vi "validate line configuration.vi"(7 "modbus":refnum<class "Modbus Module configuration.lvclass">, 11 "line in":T1) -> (1 "valid?":bool, 2 "issues":string, 3 "line out":T1)   [LabVIEW 2015, in "Modbus Module editor node.lvclass"]
doc: "Validate that Line In is a valid Modbus line and can be added to existing Configuration In without any conflicts.\n\nPlatypus Framework 1.0.1.65\nNI Systems Engineering - National Instruments"
uses:
  Modbus Module editor node.lvclass
  table line.ctl
  module/module channel/Modbus Module Channel.lvclass
  module/configuration/Modbus Module configuration.lvclass
  module/configuration/Modbus Module configuration.lvclass/Modbus Module configuration.ctl
  <vilib>/NI/Tag Bus/tag/tag descriptor.lvclass/tag descriptor.ctl
  module/module channel/Modbus Module Channel.lvclass/Modbus Module Channel.ctl
  <vilib>/NI/Tag Bus/tag/Data Type.ctl
  <vilib>/NI/Tag Bus/tag/read tag name.vi
  module/module channel/Read modbus type.vi
  module/module channel/Read starting address.vi
  <vilib>/NI/Tag Bus/tag/read data type.vi
  module/module channel/Read subindex (bool).vi
  <vilib>/NI/Tag Bus/tag/tag descriptor.lvclass
  <vilib>/NI/Tag Bus Module Framework/module configuration/TBM module configuration.lvclass
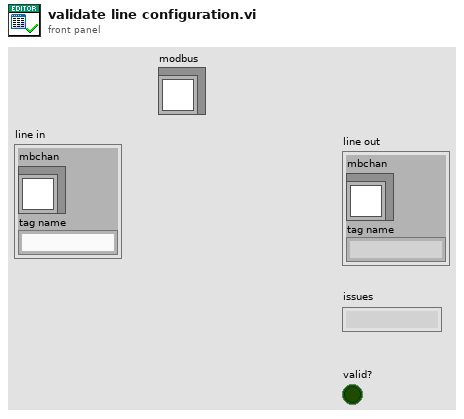
[diagram p1: front panel]
types:
  T1 = typedef "Modbus Module editor node.lvclass/table line.ctl" = cluster{"mbchan":refnum<class "Modbus Module Channel.lvclass">, "tag name":string}
  T2 = typedef "tag bus.lvlib/tag descriptor.lvclass/Data Type.ctl" = enum16{"Double", "Single", "I64", "I32", "I16", "I8", "U64", "U32", "U16", "U8", "Boolean", "String", "Array of Double", "Array of Single", "Array of I64", "Array of I32", "Array of I16", "Array of I8", "Array of U64", "Array of U32", "Array of U16", "Array of U8", "Array of Boolean", "Array of String"}
  T3 = typedef "Modbus Module Channel.lvclass/data bank type.ctl" = enum16{"Coils", "Discrete Inputs", "Input Registers", "Holding Registers"}
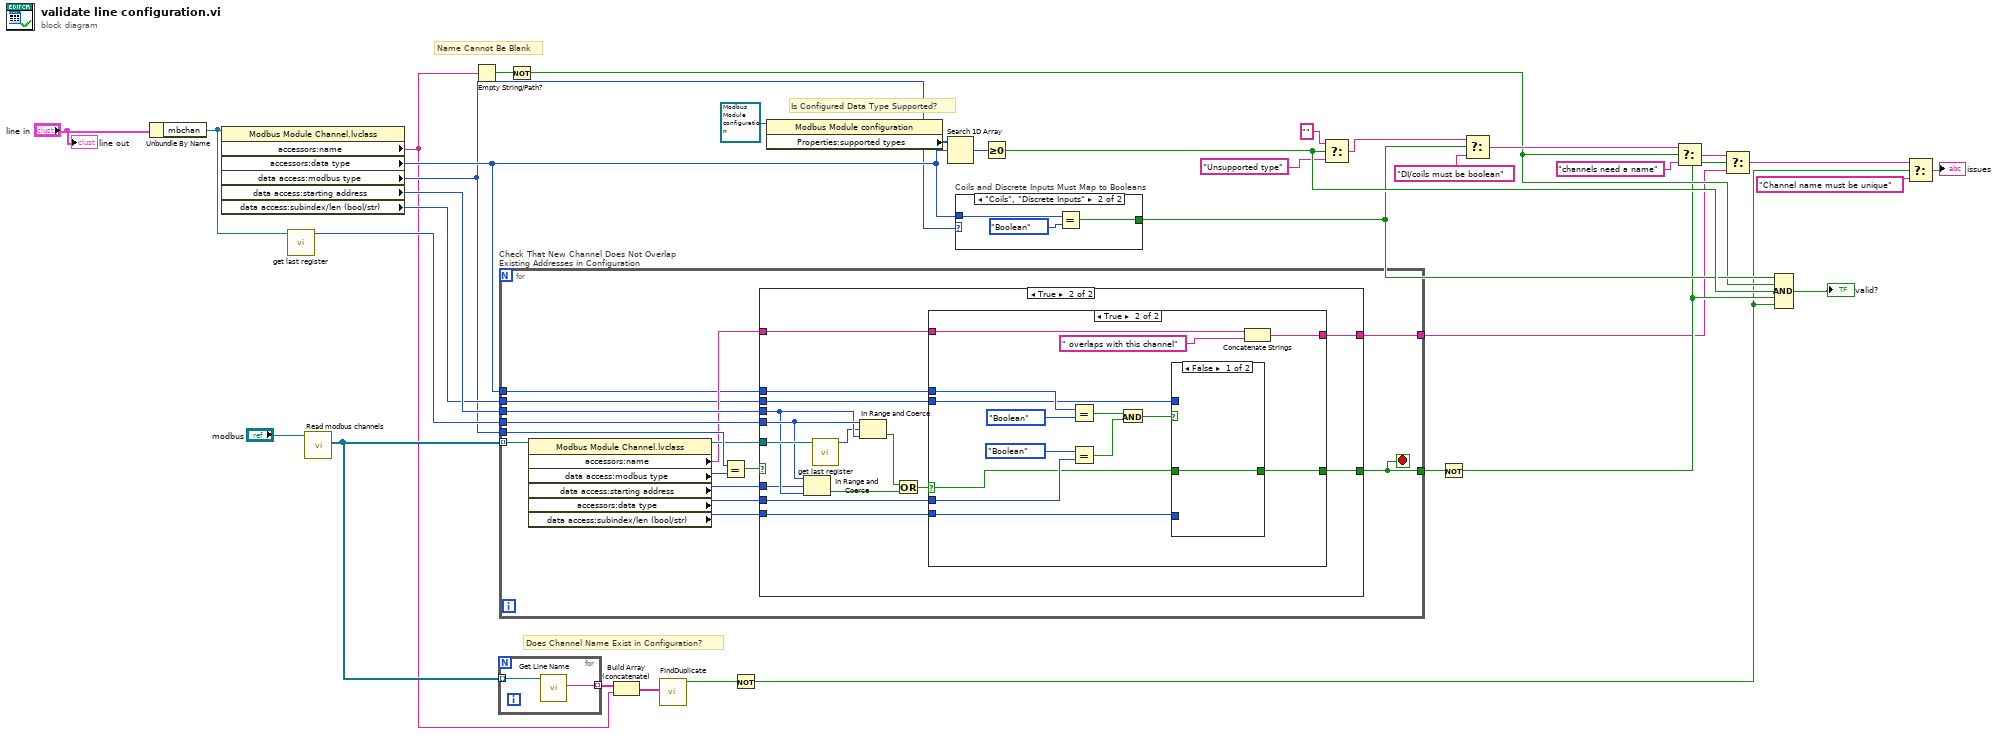
[diagram p0: block diagram]
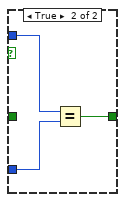
[diagram p4: hidden frame]
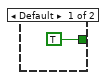
[diagram p5: hidden frame]
diagram:
  # "Does Channel Name Exist in Configuration?"
  # "Is Configured Data Type Supported?"
  # "Name Cannot Be Blank"
  n1 = Unbundle By Name("line in") -> ("mbchan"=w21:refnum<class "Modbus Module Channel.lvclass">)
  n2 = property class="Modbus Module Channel.lvclass"(reference=w21) -> ("accessors:name"=w5:string, "accessors:data type"=w12:T2, "data access:modbus type"=w11:T3, "data access:starting address"=w16:u16, "data access:subindex/len (bool/str)"=w13:i32)  [unwired: 1 in, 2 out]
  n3 = call "get last register.vi"("Modbus Module Channel in"=w21) -> ("last element"=w15:i32)  [unwired: 10 in]
  n4 = call "Read modbus channels.vi"("Modbus Slave configuration in"="modbus") -> ("modbus channels"=w7:refnum<class "Modbus Module Channel.lvclass">[])  [unwired: 8 in, 2 out]
  n5 = Empty String/Path?(string/path=w5) -> (empty?=w34:bool)
  n6 = for {
    tunnel: w7 -> [w37] mode=indexing
    tunnel: [w36] -> w6 mode=indexing
    n7 = call "Get Line Name.vi"("MB Channel"=w37) -> ("Name"=w36:string)  [unwired: 8 in, 2 out]
  }
  n8 = for "Check That New Channel Does Not Overlap Existing Addresses in Configuration" {
    tunnel: w7 -> [w52] mode=indexing
    tunnel: w11 -> [w50]
    tunnel: [w48] -> w17
    tunnel: w16 -> [w46]
    tunnel: w15 -> [w45]
    tunnel: [w43] -> w14
    tunnel: w12 -> [w40]
    tunnel: w13 -> [w38]
    stop <- w48 stop-if-true
    n9 = property class="Modbus Module Channel.lvclass"(reference=w52) -> (reference out=w47:refnum<class "Modbus Module Channel.lvclass">, "accessors:name"=w42:string, "data access:modbus type"=w51:T3, "data access:starting address"=w44:u16, "accessors:data type"=w41:T2, "data access:subindex/len (bool/str)"=w39:i32)  [unwired: 1 in, 1 out]
    n10 = Equal?(x=w50, y=w51) -> (x = y?=w49:bool)
    n11 = case shown="True" w49 {
      selector: w49 -> [w53 _]
      tunnel: [w53 w59] -> w48
      tunnel: w47 -> [_ w68]
      tunnel: w46 -> [_ w66]
      tunnel: w45 -> [_ w67]
      tunnel: w44 -> [_ w64]
      tunnel: [_ w60] -> w43
      tunnel: w42 -> [_ w58]
      tunnel: w41 -> [_ w57]
      tunnel: w40 -> [_ w56]
      tunnel: w39 -> [_ w55]
      tunnel: w38 -> [_ w54]
      frame False {
      }
      frame True {
        n12 = In Range and Coerce(upper limit=w67, x=w64, lower limit=w66) -> (In Range?=w62:bool)  [unwired: 1 out]
        n13 = call "get last register.vi"("Modbus Module Channel in"=w68) -> ("last element"=w65:i32)  [unwired: 10 in]
        n14 = In Range and Coerce(upper limit=w67, x=w65, lower limit=w66) -> (In Range?=w63:bool)  [unwired: 1 out]
        n15 = Or(x=w63, y=w62) -> (x .or. y?=w61:bool)
        n16 = case shown="True" w61 {
          selector: w61 -> [w69 w75]
          tunnel: [_ w71] -> w60
          tunnel: [w69 w76] -> w59
          tunnel: w58 -> [_ w70]
          tunnel: w57 -> [_ w83]
          tunnel: w56 -> [_ w80]
          tunnel: w55 -> [_ w74]
          tunnel: w54 -> [_ w73]
          frame False {
          }
          frame True {
            n17 = Equal?(x=w80, y=Data_Type."Boolean") -> (x = y?=w79:bool)
            n18 = Equal?(x=Data_Type."Boolean" ("y"), y=w83) -> (x = y?=w78:bool)
            n19 = And(x=w79, y=w78) -> (x .and. y?=w77:bool)
            n20 = case shown="False" w77 {
              tunnel: [w84 w85] -> w76
              tunnel: w75 -> [w84 _]
              tunnel: w74 -> [_ w86]
              tunnel: w73 -> [_ w87]
              frame False {
              }
              frame True {
                n21 = Equal?(x=w87, y=w86) -> (x = y?=w85:bool)
              }
            }
            n22 = Concatenate Strings(w70, " overlaps with this channel" ("string")) -> (w71:string)
          }
        }
      }
    }
  }
  n23 = Not(x=w34) -> (.not. x?=w23:bool)
  n24 = Build Array (concatenate)(w6, w5) -> (w4:string[])
  n25 = call <vilib>:"FindDuplicate.vi"("Array"=w4) -> ("Duplicate"=w3:bool)  [unwired: 8 in, 2 out]
  n26 = Not(x=w3) -> (.not. x?=w1:bool)
  n27 = property class="Modbus Module configuration"(reference=refnum<class "Modbus Module configuration.lvclass"> refnum ("tag bus configurable plugin module configuration")) -> ("Properties:supported types"=w32:T2[])  [unwired: 1 in, 2 out]
  n28 = Search 1D Array(1D array=w32, element=w12) -> (index of element=w30:i32)  [unwired: 1 in]
  n29 = case "Coils and Discrete Inputs Must Map to Booleans" shown="\"Coils\", \"Discrete Inputs\"" w11 {
    tunnel: [TRUE w91] -> w26
    tunnel: w12 -> [_ w90]
    frame Default {
    }
    frame "Coils", "Discrete Inputs" {
      n30 = Equal?(x=w90, y=Data_Type."Boolean") -> (x = y?=w91:bool)
    }
  }
  n31 = Greater Or Equal To 0?(x=w30) -> (x >= 0?=w29:bool)
  n32 = Select(t="", s=w29, f="Unsupported type") -> (s? t:f=w27:string)
  n33 = Not(x=w17) -> (.not. x?=w18:bool)
  n34 = Select(t=w27, s=w26, f="DI/coils must be boolean") -> (s? t:f=w24:string)
  n35 = Select(t=w24, s=w23, f="channels need a name") -> (s? t:f=w19:string)
  n36 = Select(t=w19, s=w18, f=w14) -> (s? t:f=w10:string)
  n37 = Compound Arithmetic op=AND(w26, w23, w29, w18, w1) -> (→"valid?":bool)
  n38 = Select(t=w10, s=w1, f="Channel name must be unique") -> (s? t:f=→"issues":string)
  "line out" <- "line in"
